vi "Overlay Image with Sector ROI.vi"(7 "FPGA Display Image In":T1=refnum, 8 "error in":errorcluster, 11 "FPGA Image":T1=refnum) -> (0 "error out":errorcluster, 3 "FPGA Display Image Out":T1)   [LabVIEW 2013]
uses:
  <vilib>/vision/Image Controls.llb/IMAQ Image.ctl
  Image Processing/Mask ROI FG Enum.ctl
  Globals/Average Sector Data.vi
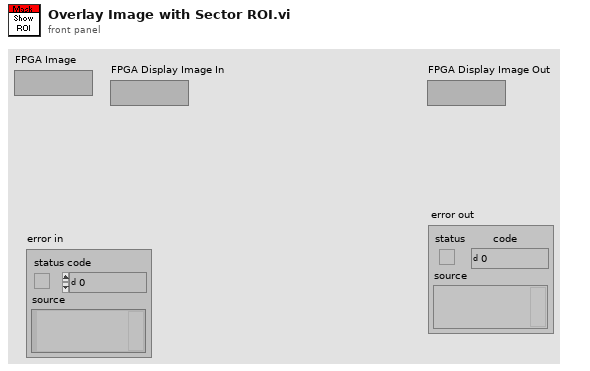
[diagram p1: front panel]
types:
  T1 = typedef "IMAQ Image.ctl" = refnum<image>
  T2 = typedef "Mask ROI FG Enum.ctl" = enum16{"Read", "Write", "Enable Background", "Disable Background"}
  T3 = typedef "Mask ROI Cluster.ctl" = cluster{"left annulus":T4, "right annulus":T4, "Threshold Range":cluster{"Lower value":dbl, "Upper value":dbl}, "[Avg BG]":u8[], "Number of Sectors":u8, "Left ROI":T5, "Right ROI":T5, "Left Start Angle Duty Cycle":fxp<+,8,0>, "Left End Angle Duty Cycle":fxp<+,8,0>, "Right End Angle Duty Cycle":fxp<+,8,0>, "Right Start Angle Duty Cycle":fxp<+,8,0>, "[Sector ROIs]":T5[]}
  T4 = typedef "IMAQ Circle" = cluster{"Center X":i32, "Center Y":i32, "Inner Radius":i32, "Outer Radius":i32, "Start Angle":dbl, "End Angle":dbl}
  T5 = typedef "ROI Descriptor" = cluster{"Global Rectangle":i32[], "Contours":cluster{"ID":enum32{"External", "Internal"}, "Type":u32, "Coordinates":i32[]}[]}
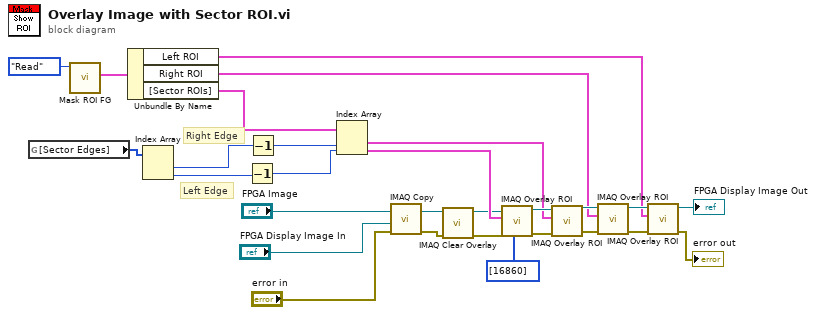
[diagram p0: block diagram]
diagram:
  # "Left Edge"
  # "Right Edge"
  n1 = global read "Average Sector Data.vi" "[Sector Edges]"() -> (w8:u8[])
  n2 = call "Mask ROI FG.vi"("Operation"=Mask_ROI_FG_Enum."Read") -> ("Mask ROI Out"=w13:T3)  [unwired: 9 in, 1 out]
  n3 = Unbundle By Name(w13) -> ("Left ROI"=w12:T5, "Right ROI"=w11:T5, "[Sector ROIs]"=w10:T5[])
  n4 = Index Array(array=w8) -> (element #1=w6:u8, element #2=w7:u8)  [unwired: 2 in]
  n5 = Decrement(x=w7) -> (x-1=w22:u8)
  n6 = Decrement(x=w6) -> (x-1=w23:u8)
  n7 = Index Array(array=w10, index #1=w23, index #2=w22) -> (element #1=w14:T5, element #2=w15:T5)
  n8 = call "IMAQ Copy"("error in (no error)"="error in", "Image Dst"="FPGA Display Image In", "Image Src"="FPGA Image") -> ("error out"=w3:errorcluster, "Image Dst Out"=w4:T1)  [unwired: 3 in]
  n9 = call "IMAQ Clear Overlay"("error in (no error)"=w3, "Image"=w4) -> ("error out"=w1:errorcluster, "Image Out"=w2:T1)  [unwired: 8 in]
  n10 = call "IMAQ Overlay ROI"("Colors (Green)"=u32[] [16860], "error in (no error)"=w1, "ROI Descriptor"=w15, "Image"=w2) -> ("error out"=w28:errorcluster, "Image Out"=w27:T1)  [unwired: 6 in]
  n11 = call "IMAQ Overlay ROI"("error in (no error)"=w28, "ROI Descriptor"=w14, "Image"=w27) -> ("error out"=w16:errorcluster, "Image Out"=w20:T1)  [unwired: 7 in]
  n12 = call "IMAQ Overlay ROI"("error in (no error)"=w16, "ROI Descriptor"=w11, "Image"=w20) -> ("error out"=w21:errorcluster, "Image Out"=w19:T1)  [unwired: 7 in]
  n13 = call "IMAQ Overlay ROI"("error in (no error)"=w21, "ROI Descriptor"=w12, "Image"=w19) -> ("error out"=→"error out":errorcluster, "Image Out"=→"FPGA Display Image Out":T1)  [unwired: 7 in]
